vi "Get All Projects.vi"(7 "Project Store in":refnum<class "Project Store.lvclass">, 8 "error in (no error)":errorcluster, 11 "include inactive?":bool) -> (0 "error out":errorcluster, 3 "Projects":T1, 5 "Project Store out":refnum<class "Project Store.lvclass">)   [LabVIEW 2024, in "Project Store.lvclass"]
doc: "Returns the projects of the in-memory model sorted by Sort Order. Inactive projects are left out unless include inactive? is TRUE.\n\nGenerated by: Claude"
uses:
  Project Store.lvclass
  Project Store.lvclass/Project Store.ctl
  Rows/Project.ctl
  Rows/Project List.ctl
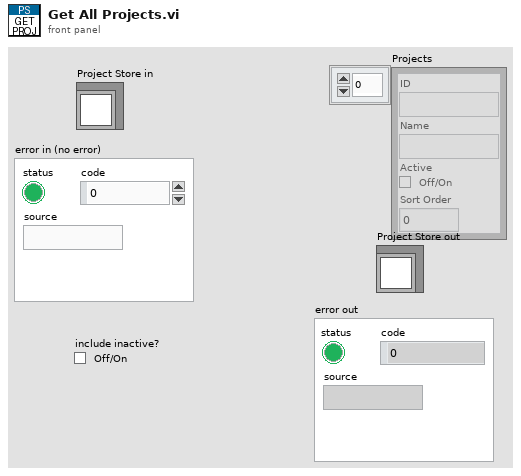
[diagram p1: front panel]
types:
  T1 = typedef "Project List.ctl" = T2[]
  T2 = typedef "Project.ctl" = cluster{"ID":string, "Name":string, "Active":bool, "Sort Order":i32}
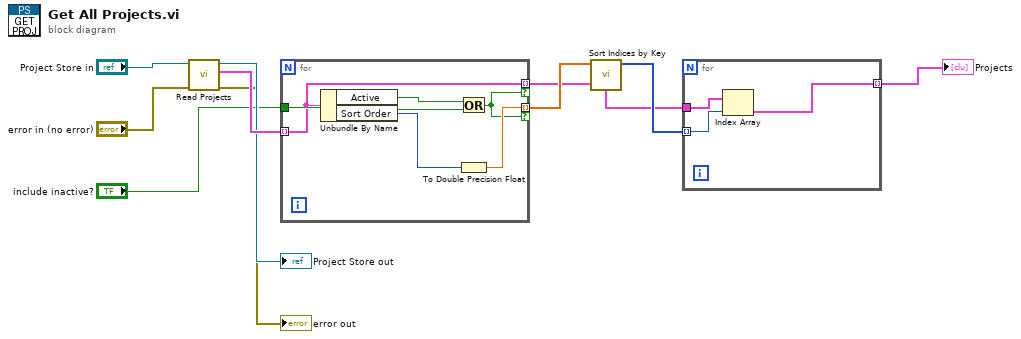
[diagram p0: block diagram]
diagram:
  n1 = call-dynamic "Read Projects.vi"("error in (no error)"="error in (no error)", "Project Store in"="Project Store in") -> ("error out"=→"error out":errorcluster, "Project List"=w6:T1, "Project Store out"=→"Project Store out":refnum<class "Project Store.lvclass">)  [unwired: 7 in]
  n2 = for {
    tunnel: "include inactive?" -> [w12]
    tunnel: w6 -> [w11] mode=indexing
    tunnel: [w11] -> w7 mode=indexing if=w15
    tunnel: [w16] -> w8 mode=indexing if=w15
    n3 = Unbundle By Name(w11) -> ("Active"=w13:bool, "Sort Order"=w14:i32)
    n4 = Or(x=w13, y=w12) -> (x .or. y?=w15:bool)
    n5 = To Double Precision Float(number=w14) -> (double precision float=w16:dbl)
  }
  n6 = call "Sort Indices by Key.vi"("Keys"=w8) -> ("Sorted Indices"=w9:i32[])  [unwired: 9 in, 1 out]
  n7 = for {
    tunnel: w7 -> [w18]
    tunnel: w9 -> [w17] mode=indexing
    tunnel: [w19] -> w10 mode=indexing
    n8 = Index Array(array=w18, index=w17) -> (element=w19:T2)
  }
  "Projects" <- w10
